vi "H11_TDMS_per_sample.vi"() -> ()   [LabVIEW 2018]
doc: "Use this template to build a VI to use as a subVI."
panel:
  out "read error":errorcluster
  out "T3 samples read":i32
  out "last i":i32
  out "error out":errorcluster
  in  "defragment after?":bool
  in  "tdms file":path
  in  "samples per channel":i32
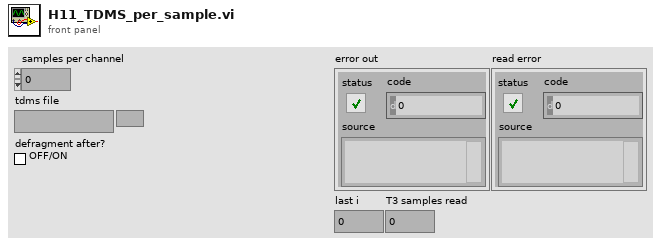
[diagram p1: front panel]
types:
  T1 = enum16{"open", "open or create", "create or replace", "create", "open (read-only)"}
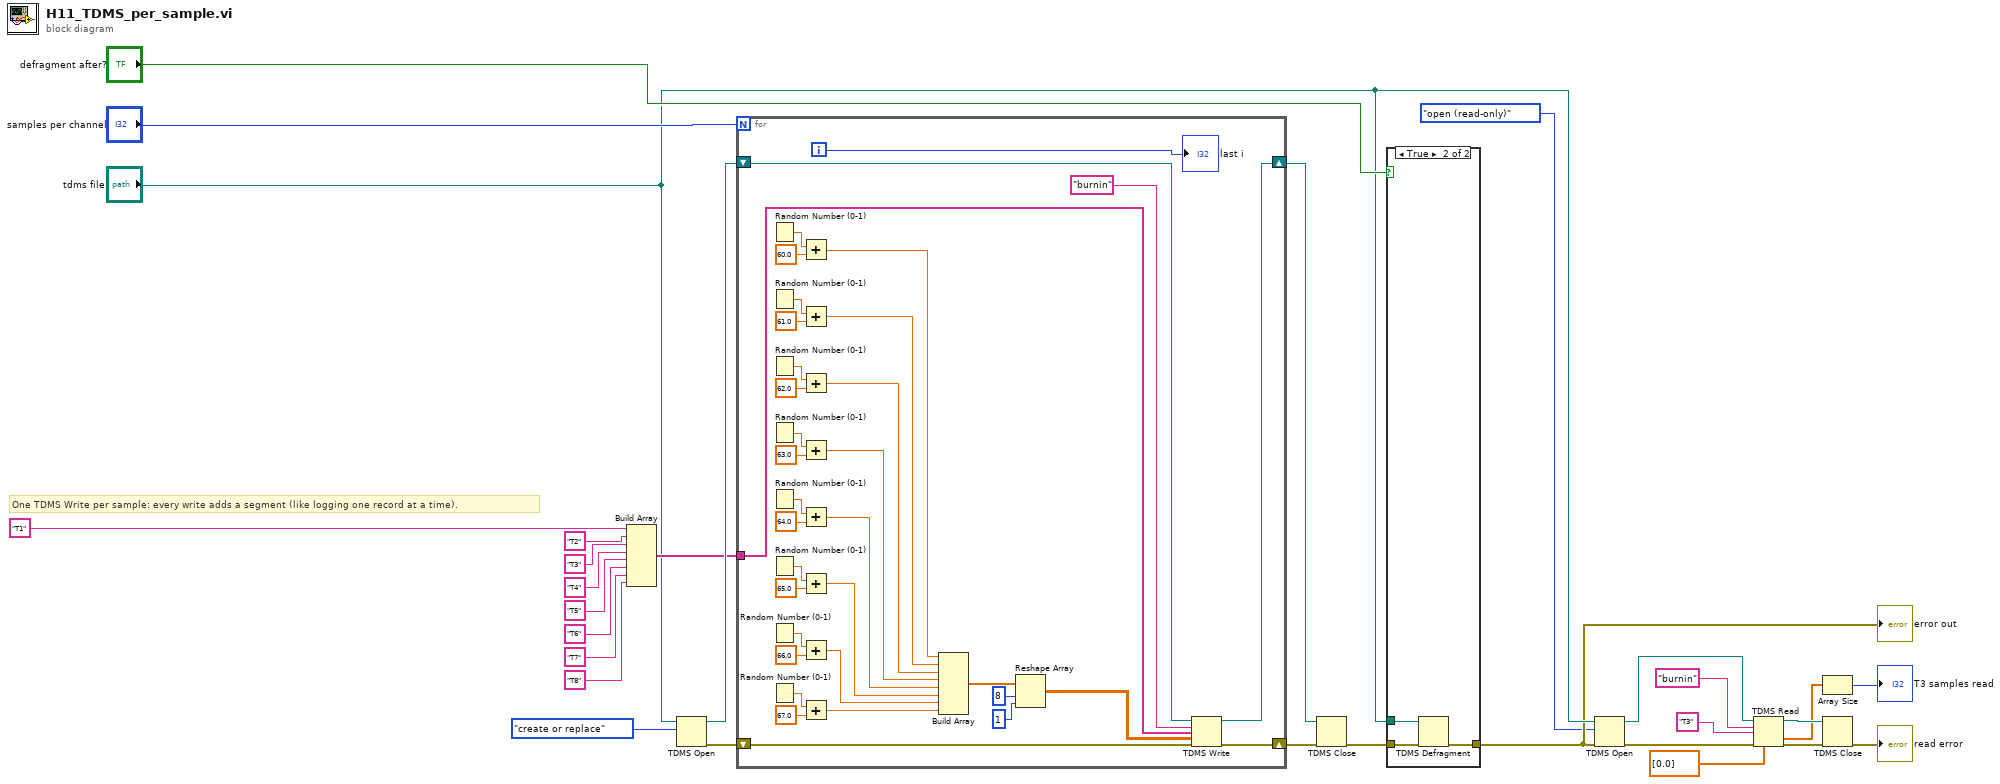
[diagram p0: block diagram]
diagram:
  # "One TDMS Write per sample: every write adds a segment (like logging one record at a time)."
  n1 = Build Array("T1", "T2", "T3", "T4", "T5", "T6", "T7", "T8") -> (w18:string[])
  n2 = TDMS Open(10:T1."create or replace" ("operation (0:open)"), 11:"tdms file") -> (0:w19:errorcluster, 3:w20:refnum<k34>)  [unwired: 5 in]
  n3 = for {
    N: "samples per channel" -> [_]
    shift-right: [w33] -> w17
    shift-left: w20 -> [w41]
    shift-right: [w32] -> w16
    shift-left: w19 -> [w40]
    tunnel: w18 -> [w38]
    i -> [w31]
    n4 = Random Number (0-1)() -> (number: 0 to 1=w65:dbl)
    n5 = Random Number (0-1)() -> (number: 0 to 1=w63:dbl)
    n6 = Random Number (0-1)() -> (number: 0 to 1=w61:dbl)
    n7 = Random Number (0-1)() -> (number: 0 to 1=w59:dbl)
    n8 = Random Number (0-1)() -> (number: 0 to 1=w57:dbl)
    n9 = Random Number (0-1)() -> (number: 0 to 1=w55:dbl)
    n10 = Random Number (0-1)() -> (number: 0 to 1=w53:dbl)
    n11 = Random Number (0-1)() -> (number: 0 to 1=w51:dbl)
    n12 = Add(x=w65, y=60.0) -> (x+y=w49:dbl)
    n13 = Add(x=w63, y=61.0) -> (x+y=w48:dbl)
    n14 = Add(x=w61, y=62.0) -> (x+y=w47:dbl)
    n15 = Add(x=w59, y=63.0) -> (x+y=w46:dbl)
    n16 = Add(x=w57, y=64.0) -> (x+y=w45:dbl)
    n17 = Add(x=w55, y=65.0) -> (x+y=w44:dbl)
    n18 = Add(x=w53, y=66.0) -> (x+y=w43:dbl)
    n19 = Add(x=w51, y=67.0) -> (x+y=w42:dbl)
    n20 = Build Array(w49, w48, w47, w46, w45, w44, w43, w42) -> (w37:dbl[])
    n21 = Reshape Array(w37, 8 ("dimension size"), 1 ("dimension size")) -> (w34:dbl[][])
    n22 = TDMS Write(0:w41, 5:"burnin", 7:w38, 9:w34, 11:w40) -> (4:w33:refnum<k34>, 15:w32:errorcluster)  [unwired: 1 in, 2 out]
    "last i" <- w31
  }
  n23 = TDMS Close(8:w16, 11:w17) -> (0:w13:errorcluster)  [unwired: 1 out]
  n24 = case shown="True" "defragment after?" {
    tunnel: "tdms file" -> [_ w69]
    tunnel: w13 -> [w66 w68]
    tunnel: [w66 w67] -> w12
    frame False {
    }
    frame True {
      n25 = TDMS Defragment(4:w68, 7:w69) -> (0:w67:errorcluster)
    }
  }
  "error out" <- w12
  n26 = TDMS Open(8:w12, 10:T1."open (read-only)" ("operation (0:open)"), 11:"tdms file") -> (0:w9:errorcluster, 3:w10:refnum<k34>)  [unwired: 4 in]
  n27 = TDMS Read(0:w10, 5:"burnin", 7:"T3", 11:w9, 12:dbl[] [0.0] ("Y")) -> (4:w5:refnum<k34>, 10:w3:dbl[], 15:w4:errorcluster)  [unwired: 3 in, 3 out]
  n28 = Array Size(array=w3) -> (size(s)=→"T3 samples read":i32)
  n29 = TDMS Close(8:w4, 11:w5) -> (0:→"read error":errorcluster)  [unwired: 1 out]
